vi "Motor stop_X(SubVI).vi"(0 "Motor, C":i32, 5 "Motor, I":i32, 7 "i":i32, 9 "Stop number":dbl, 11 "Stop number_L":refnum<vi>) -> (4 "Motor, O":i32, 6 "Loop stop":bool, 8 "up":bool, 10 "left":bool)   [LabVIEW 2018]
panel:
  out "Numeric":dbl
  out "i":dbl
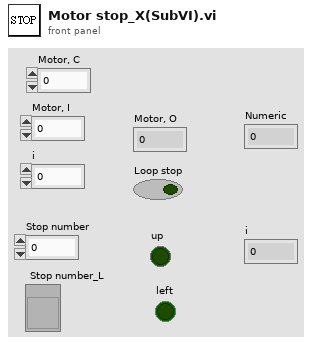
[diagram p1: front panel]
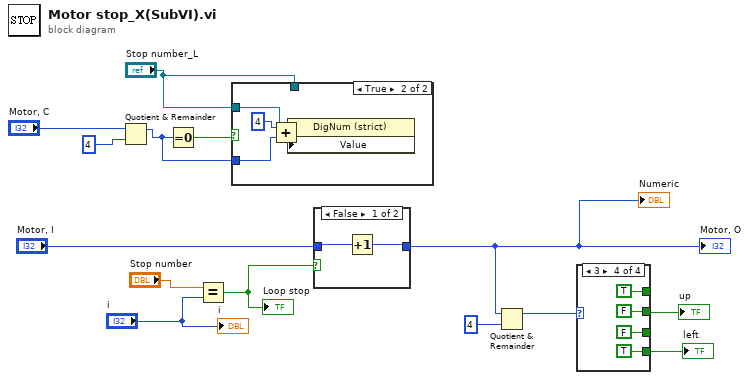
[diagram p0: block diagram]
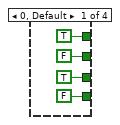
[diagram p2: hidden frame]
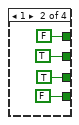
[diagram p3: hidden frame]
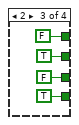
[diagram p4: hidden frame]
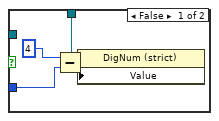
[diagram p5: hidden frame]
diagram:
  n1 = Quotient & Remainder(x="Motor, C", y=4) -> (x-y*floor(x/y)=w13:i32)  [unwired: 1 out]
  n2 = Equal To 0?(x=w13) -> (x = 0?=w8:bool)
  n3 = Equal?(x="Stop number", y="i") -> (x = y?=w14:bool)
  "Loop stop" <- w14
  n4 = case shown="True" w8 {
    tunnel: w13 -> [w18 w20]
    tunnel: "Stop number_L" -> [w15 _]
    tunnel: "Stop number_L" -> [_ w19]
    frame False {
      n5 = Subtract(x=4, y=w18) -> (x-y=w16:i32)
      n6 = property class="DigNum (strict)"(reference=w15, "Value"=w16) -> ()  [unwired: 1 in, 2 out]
    }
    frame True {
      n7 = Add(x=4, y=w20) -> (x+y=w21:i32)
      n8 = property class="DigNum (strict)"(reference=w19, "Value"=w21) -> ()  [unwired: 1 in, 2 out]
    }
  }
  n9 = case shown="False" w14 {
    tunnel: "Motor, I" -> [w24 w25]
    tunnel: [w23 w25] -> w3
    frame False {
      n10 = Increment(x=w24) -> (x+1=w23:i32)
    }
    frame True {
    }
  }
  "Numeric" <- w3
  "Motor, O" <- w3
  n11 = Quotient & Remainder(x=w3, y=4) -> (x-y*floor(x/y)=w4:i32)  [unwired: 1 out]
  n12 = case shown="3" w4 {
    tunnel: [FALSE FALSE TRUE TRUE] -> w1
    tunnel: [TRUE TRUE FALSE FALSE] -> _
    tunnel: [FALSE TRUE TRUE FALSE] -> w2
    tunnel: [TRUE FALSE FALSE TRUE] -> _
    frame 0, Default {
    }
    frame 1 {
    }
    frame 2 {
    }
    frame 3 {
    }
  }
  "up" <- w2
  "left" <- w1
  "i" <- "i"
